vi "CCT_simple_example.vi"() -> ()   [LabVIEW 2019]
uses:
  TLCCT.lvlib
  C:/Users/gboedecker/OneDrive - THORLABS Inc/Documents/cct_test/LabView/net462/Thorlabs.ManagedDevice.CompactSpectrographDriver.dll
  net462/Thorlabs.ManagedDevice.CompactSpectrographDriver.dll
  DeviceManager/TLCCT_StartupHelper.ctl
panel:
  in  "Target Exposure [ms]":sgl=1.0 min=0.01 max=60000 format="%#.2f"
  out "Last acquired Spectrum":cluster{"X":dbl, "Y":dbl}[](graph) caption="Timestamp: 11:35:43.332"
  out "error out":errorcluster
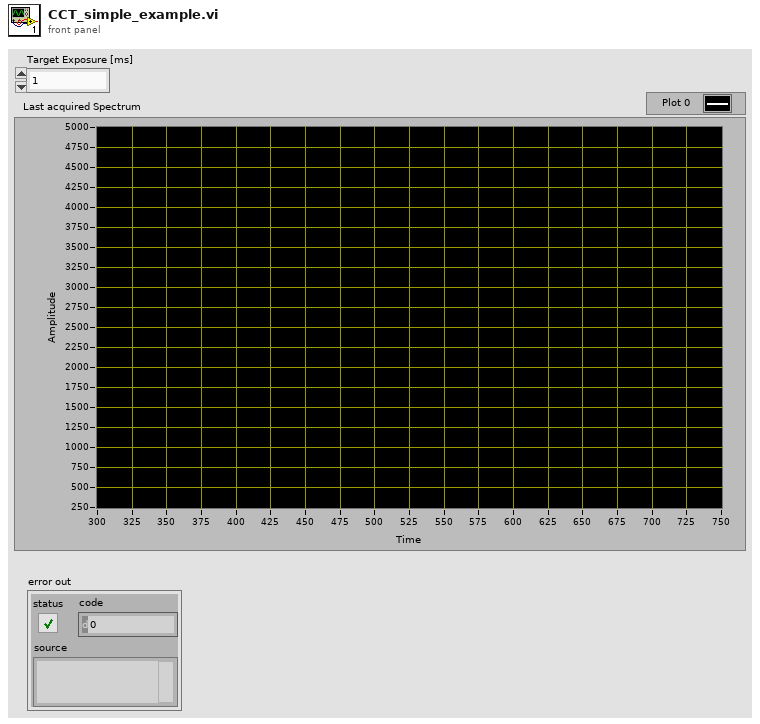
[diagram p1: front panel]
types:
  T1 = typedef "TLCCT.lvlib/TLCCT_StartupHelper.ctl" = cluster{"Library Installed":bool, "LibraryPath":path, "Startup Helper":refnum<k24>, "CancellationToken":refnum<k24>, "Managed Spectrometer":cluster{"Device ID":string, "CancellationToken":refnum<k24>, "Spectrometer\nHandle":refnum<k24>}}
  T2 = cluster{"Device ID":string, "CancellationToken":refnum<k24>, "Spectrometer\nHandle":refnum<k24>}
  T3 = typedef "TLCCT.lvlib/TLCCT_Spectrum.ctl" = cluster{"Intensity":dbl[], "Wavelength":dbl[], "Acquired":timestamp, "Sensor Exposure, ms":sgl, "Hardware Average, Frames":i32, "Trigger Mode":bool, "Tick":u64, "Amplitude Corrected":bool}
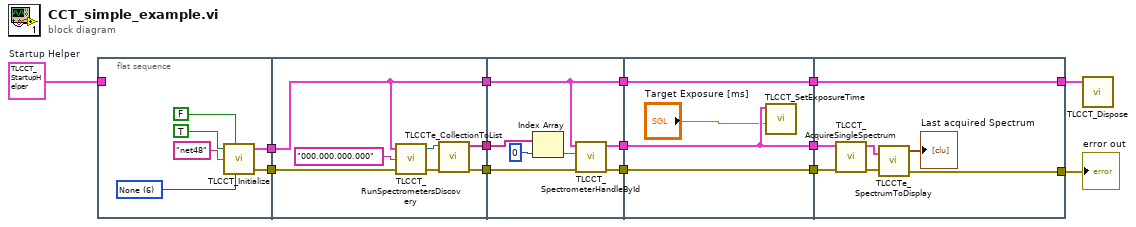
[diagram p0: block diagram]
diagram:
  w12 = T1 {"Library Installed"=FALSE, "LibraryPath"=path "", "Startup Helper"=refnum, "CancellationToken"=refnum, "Managed Spectrometer"={"Device ID"="", "CancellationToken"=refnum, "Spectrometer\nHandle"=refnum}}  # Startup Helper
  n1 = flat-sequence {
    tunnel: [w17] -> w14
    tunnel: w12 -> [_]
    tunnel: [w16] -> w11
    tunnel: w14 -> [w21]
    tunnel: [w21] -> w13
    tunnel: w11 -> [w26]
    tunnel: [w24] -> w9
    tunnel: [w23] -> w8
    tunnel: w13 -> [w28]
    tunnel: [w28] -> w4
    tunnel: w9 -> [w34]
    tunnel: [w33] -> w6
    tunnel: [w29] -> w2
    tunnel: w8 -> [w32]
    tunnel: w6 -> [w38]
    tunnel: [w38] -> w5
    tunnel: w4 -> [w37]
    tunnel: [w37] -> w3
    tunnel: w2 -> [w36]
    tunnel: [w36] -> w1
    tunnel: [w40] -> w10
    tunnel: w5 -> [w41]
    tunnel: w3 -> [w40]
    tunnel: w1 -> [w39]
    tunnel: [w42] -> w7
    frame #0 {
      w18 = 6 items=["Trace", "Debug", "Information", "Warning", "Error", "Critical", "None"] ("Log Level")
      n2 = call "TLCCT_Initialize.vi"("Location Check"=TRUE, "With Virtual Device"=FALSE, "DLL Source"="net48", "Log Level"=w18) -> ("Data"=w17:T1, "Error Out"=w16:errorcluster)  [unwired: 1 in, 1 out]
    }
    frame #1 {
      n3 = call "TLCCT_RunSpectrometersDiscovery.vi"("Error In"=w26, "IP Address"="000.000.000.000" ("Target IP"), "Startup Helper"=w21) -> ("Error Out"=w25:errorcluster, "Known Spectrometers"=w27:refnum<k24>)  [unwired: 1 in]
      n4 = call "TLCCTe_CollectionToList.vi"("Error In"=w25, "Collection"=w27) -> ("Error Out"=w24:errorcluster, "List"=w23:string[])  [unwired: 3 in, 2 out]
    }
    frame #2 {
      n5 = Index Array(array=w32, index=0) -> (element=w30:string)
      n6 = call "TLCCT_SpectrometerHandleById.vi"("Error In"=w34, "Spectrometer ID"=w30, "Startup Helper"=w28) -> ("Error Out"=w33:errorcluster, "Managed Spectrometer"=w29:T2)  [unwired: 1 in, 3 out]
    }
    frame #3 {
      n7 = call "TLCCT_SetExposureTime.vi"("Target Exposure, ms"="Target Exposure [ms]", "Managed Spectrometer"=w36) -> ()  [unwired: 2 in, 3 out]
    }
    frame #4 {
      n8 = call "TLCCT_AcquireSingleSpectrum.vi"("Error In"=w41, "Managed Spectrometer"=w39) -> ("Error Out"=w45:errorcluster, "Acquired Spectrum"=w44:T3)  [unwired: 2 in, 2 out]
      n9 = call "TLCCTe_SpectrumToDisplay.vi"("Spectrum"=w44, "Error In"=w45) -> ("Last acquired Spectrum"=→"Last acquired Spectrum":cluster{"X":dbl, "Y":dbl}[], "Error Out"=w42:errorcluster)  [unwired: 1 out]
    }
  }
  n10 = call "TLCCT_Dispose.vi"("Startup Helper"=w10) -> ()  [unwired: 4 in, 1 out]
  "error out" <- w7
